vi "sync init all semaphores.vi"(8 "error in (no error)":errorcluster, 10 "pointer to shared memory":u64, 11 "sync items":T3[](array[typedef])) -> (0 "error out":errorcluster, 2 "offset pointer out":u64, 3 "initialized semaphores":T1[](array[typedef]))   [LabVIEW 2014, in "Shared Memory runtime.lvclass"]
uses:
  Shared Memory runtime.lvclass
  editor node/sync/sync item.ctl
  editor node/sync/sync mechanism.ctl
  controls/semaphore data.ctl
  <vilib>/NI/NI Linux RT IPC/POSIX Threads/Classes/Semaphore/Controls/reference.ctl
  <vilib>/NI/NI Linux RT IPC/POSIX Threads/Classes/Semaphore/Semaphore.lvclass
  configuration/Shared Memory configuration.lvclass
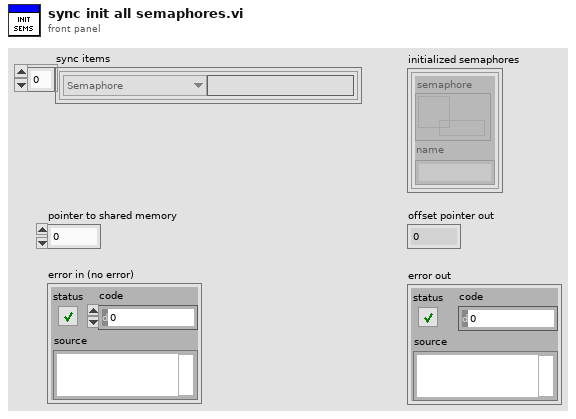
[diagram p1: front panel]
types:
  T1 = typedef "Shared Memory runtime.lvclass/semaphore data.ctl" = cluster{"semaphore":T2, "name":string}
  T2 = typedef "Linux RT IPC.POSIX Threads.lvlib/Semaphore.lvclass/reference.ctl" = refnum<data-value>
  T3 = typedef "Shared Memory configuration.lvclass/sync item.ctl" = cluster{"mechanism":T4, "name":string}
  T4 = typedef "Shared Memory configuration.lvclass/sync mechanism.ctl" = enum16{"Semaphore"}
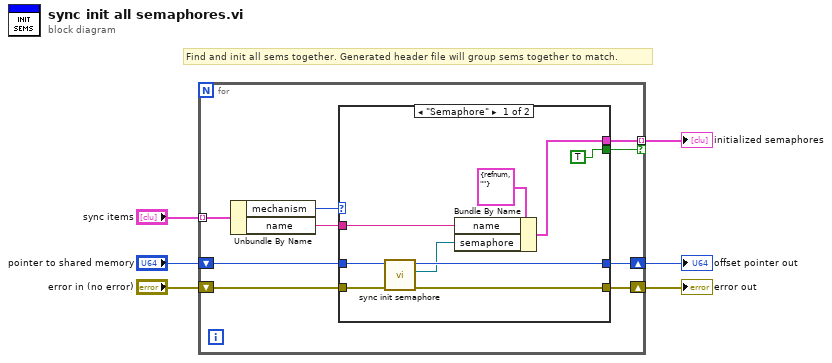
[diagram p0: block diagram]
diagram:
  # "Find and init all sems together. Generated header file will group sems together to match."
  n1 = for {
    tunnel: "sync items" -> [w15] mode=indexing
    shift-right: [w10] -> w3
    shift-left: "pointer to shared memory" -> [w11]
    shift-right: [w9] -> w2
    shift-left: "error in (no error)" -> [w12]
    tunnel: [w8] -> w1 mode=indexing if=w7
    n2 = Unbundle By Name(w15) -> ("mechanism"=w14:T4, "name"=w13:string)
    n3 = case shown="\"Semaphore\"" w14 {
      tunnel: [w17 _] -> w8
      tunnel: w13 -> [w20 _]
      tunnel: w12 -> [w23 w26]
      tunnel: w11 -> [w22 w25]
      tunnel: [w21 w25] -> w10
      tunnel: [w18 w26] -> w9
      tunnel: [TRUE _] -> w7
      frame "Semaphore" {
        n4 = call "sync init semaphore.vi"("error in (no error)"=w23, "pointer in"=w22) -> ("error out"=w18:errorcluster, "Semaphore out"=w19:T2, "offset pointer out"=w21:u64)  [unwired: 7 in]
        n5 = Bundle By Name(cluster=T1 {"semaphore"=refnum, "name"=""} ("semaphore data"), "name"=w20, "semaphore"=w19) -> (w17:T1)
      }
      frame Default {
      }
    }
  }
  "initialized semaphores" <- w1
  "offset pointer out" <- w3
  "error out" <- w2
